vi "After Run TS.vi"(8 "error in":errorcluster, 11 "Heat Flow Test Stand in":refnum<class "Heat Flow Test Stand.lvclass">) -> (0 "error out":errorcluster, 3 "Heat Flow Test Stand out":refnum<class "Heat Flow Test Stand.lvclass">)   [LabVIEW 2019, in "Test Stands.lvlib" / "Heat Flow Test Stand.lvclass"]
uses:
  Heat Flow Test Stand.lvclass
  C:/Users/wg/Documents/LV_Projects/test-stand/App/Generic Test Stand/Generic Test Stand.lvclass
  DAC/Heat Flow/HeatFlow AIV/DAC HeatFlow AIV.lvclass
  C:/Users/wg/Documents/LV_Projects/test-stand/App/DAC/DAC.lvclass
  Generic Test Stand/Generic Test Stand.lvclass/Generic Test Stand.ctl
  Heat Flow Test Stand.lvclass/Heat Flow Test Stand.ctl
  DAC/DAC.lvclass/DAC.ctl
  DAC/DAC.lvclass
  Generic Test Stand/Generic Test Stand.lvclass
  DAC/Heat Flow/HeatFlow AOV/DAC HeatFlow AOV.lvclass
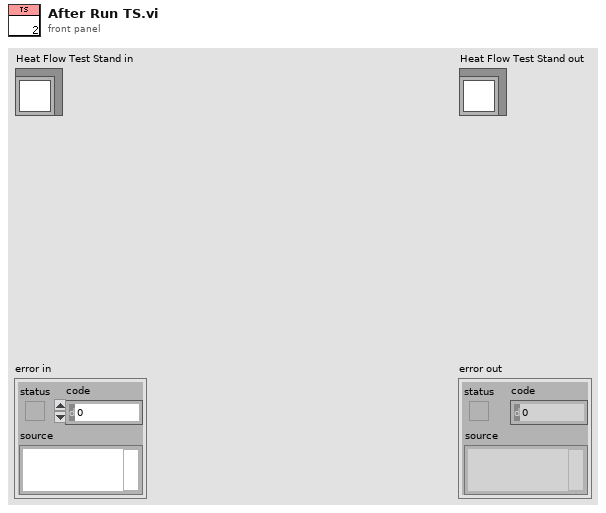
[diagram p1: front panel]
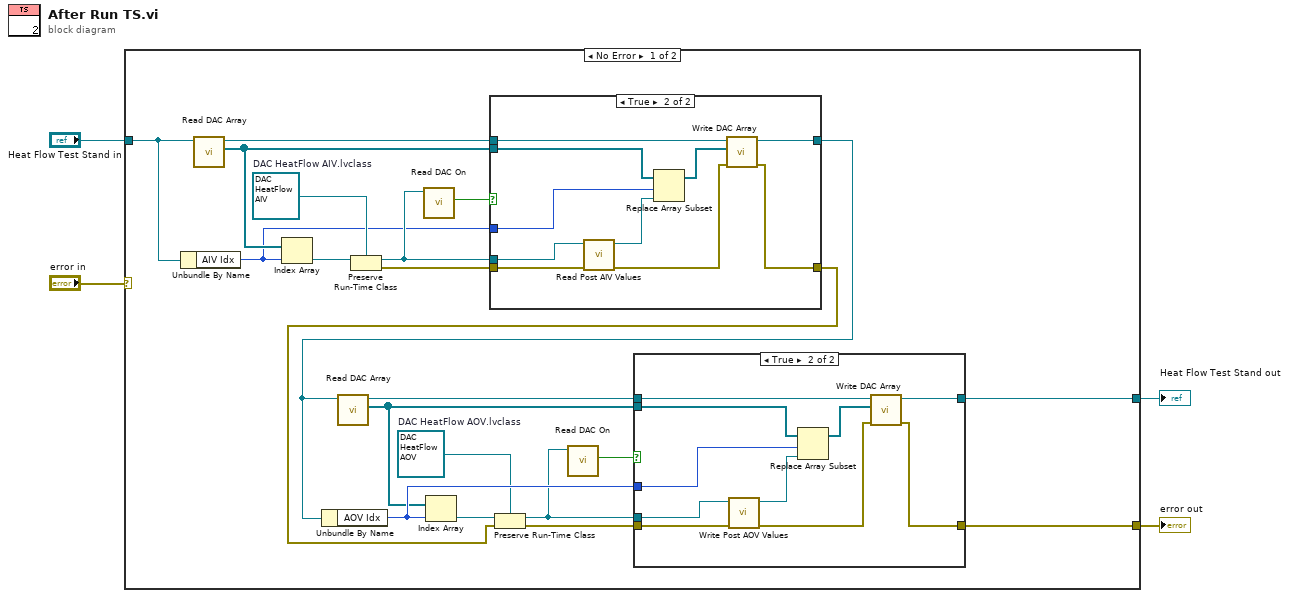
[diagram p0: block diagram]
diagram:
  n1 = case shown="No Error" "error in" {
    selector: "error in" -> [_ w51]
    tunnel: [w6 w51] -> w1
    tunnel: [w7 w50] -> w2
    tunnel: "Heat Flow Test Stand in" -> [w20 w50]
    frame No Error {
      w5 = refnum<class "DAC HeatFlow AOV.lvclass"> refnum  # DAC HeatFlow AOV.lvclass
      w19 = refnum<class "DAC HeatFlow AIV.lvclass"> refnum  # DAC HeatFlow AIV.lvclass
      n2 = Unbundle By Name(w20) -> ("AIV Idx"=w17:i32)
      n3 = call "Read DAC Array.vi"("Generic Test Stand in"=w20) -> ("DAC Array"=w21:refnum<class "DAC.lvclass">[], "Generic Test Stand out"=w24:refnum<class "Heat Flow Test Stand.lvclass">)  [unwired: 8 in, 1 out]
      n4 = Index Array(array=w21, index=w17) -> (element=w23:refnum<class "DAC.lvclass">)
      n5 = Preserve Run-Time Class(object in=w23, 2:w19) -> (object out=w18:refnum<class "DAC HeatFlow AIV.lvclass">, error out=w22:errorcluster)  [unwired: 1 in]
      n6 = call "Read DAC On.vi"("DAC in"=w18) -> ("DAC On"=w25:bool)  [unwired: 8 in, 2 out]
      n7 = case shown="True" w25 {
        tunnel: w24 -> [w39 w47]
        tunnel: [w39 w49] -> w9
        tunnel: w18 -> [_ w43]
        tunnel: w22 -> [w38 w44]
        tunnel: w21 -> [_ w48]
        tunnel: [w38 w45] -> w8
        tunnel: w17 -> [_ w40]
        frame False {
        }
        frame True {
          n8 = call "Read Post AIV Values.vi"("error in"=w44, "DAC HeatFlow AIV in"=w43) -> ("error out"=w41:errorcluster, "DAC HeatFlow AIV out"=w42:refnum<class "DAC HeatFlow AIV.lvclass">)  [unwired: 8 in]
          n9 = Replace Array Subset(array=w48, new element=w42, index=w40) -> (w46:refnum<class "DAC.lvclass">[])
          n10 = call "Write DAC Array.vi"("error in (no error)"=w41, "DAC Array"=w46, "Generic Test Stand in"=w47) -> ("error out"=w45:errorcluster, "Generic Test Stand out"=w49:refnum<class "Heat Flow Test Stand.lvclass">)  [unwired: 7 in]
        }
      }
      n11 = Unbundle By Name(w9) -> ("AOV Idx"=w16:i32)
      n12 = call "Read DAC Array.vi"("Generic Test Stand in"=w9) -> ("DAC Array"=w14:refnum<class "DAC.lvclass">[], "Generic Test Stand out"=w11:refnum<class "Heat Flow Test Stand.lvclass">)  [unwired: 8 in, 1 out]
      n13 = Index Array(array=w14, index=w16) -> (element=w12:refnum<class "DAC.lvclass">)
      n14 = Preserve Run-Time Class(object in=w12, error in=w8, 2:w5) -> (object out=w15:refnum<class "DAC HeatFlow AOV.lvclass">, error out=w13:errorcluster)
      n15 = call "Read DAC On.vi"("DAC in"=w15) -> ("DAC On"=w10:bool)  [unwired: 8 in, 2 out]
      n16 = case shown="True" w10 {
        tunnel: w11 -> [w27 w35]
        tunnel: [w27 w37] -> w7
        tunnel: w15 -> [_ w30]
        tunnel: w13 -> [w26 w31]
        tunnel: w14 -> [_ w36]
        tunnel: [w26 w33] -> w6
        tunnel: w16 -> [_ w32]
        frame False {
        }
        frame True {
          n17 = call "Write Post AOV Values.vi"("error in"=w31, "DAC HeatFlow AOV in"=w30) -> ("error out"=w28:errorcluster, "DAC HeatFlow AOV out"=w29:refnum<class "DAC HeatFlow AOV.lvclass">)  [unwired: 8 in]
          n18 = Replace Array Subset(array=w36, new element=w29, index=w32) -> (w34:refnum<class "DAC.lvclass">[])
          n19 = call "Write DAC Array.vi"("error in (no error)"=w28, "DAC Array"=w34, "Generic Test Stand in"=w35) -> ("error out"=w33:errorcluster, "Generic Test Stand out"=w37:refnum<class "Heat Flow Test Stand.lvclass">)  [unwired: 7 in]
        }
      }
    }
    frame Error {
    }
  }
  "error out" <- w1
  "Heat Flow Test Stand out" <- w2
